vi "FilterResults.vi"(8 "error in (no error)":errorcluster, 11 "CDependencyInspection in":refnum<class "CDependencyInspection.lvclass">) -> (0 "error out":errorcluster, 3 "CDependencyInspection out":refnum<class "CDependencyInspection.lvclass">)   [LabVIEW 2020, in "DependencyInspection.lvlib" / "CDependencyInspection.lvclass"]
uses:
  CDependencyInspection.lvclass
  CDependencyList/CDependencyList.lvclass
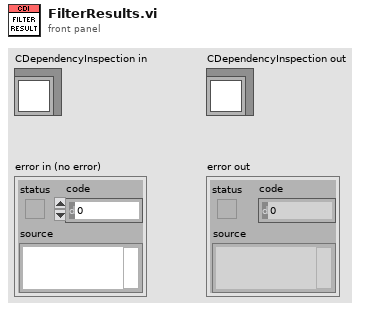
[diagram p1: front panel]
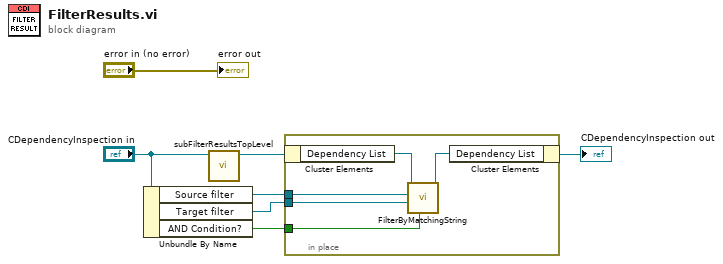
[diagram p0: block diagram]
diagram:
  n1 = Unbundle By Name("CDependencyInspection in") -> ("Source filter"=w3:refnum<class "CItemMatch.lvclass">, "Target filter"=w2:refnum<class "CItemMatch.lvclass">, "AND Condition?"=w1:bool)
  n2 = call "subFilterResultsTopLevel.vi"("CDependencyInspection in"="CDependencyInspection in") -> ("CDependencyInspection out"=w6:refnum<class "CDependencyInspection.lvclass">)  [unwired: 9 in, 1 out]
  n3 = in-place {
    in-place-border: w3 -> [w11]
    in-place-border: w2 -> [w10]
    in-place-border: w1 -> [w8]
    n4 = in-place-cluster #1(w6) -> ("Dependency List"=w9:refnum<class "CDependencyList.lvclass">)
    n5 = call-dynamic "FilterByMatchingString.vi"("AND Condition?"=w8, "Target filter"=w10, "Source filter"=w11, "CDependencyList in"=w9) -> ("CDependencyList out"=w12:refnum<class "CDependencyList.lvclass">)  [unwired: 6 in, 1 out]
    n6 = in-place-cluster #1("Dependency List"=w12) -> (→"CDependencyInspection out":refnum<class "CDependencyInspection.lvclass">)
  }
  "error out" <- "error in (no error)"
